vi "GO alertes Keller.vi"(5 "Numéro":u8) -> ()   [LabVIEW 2022 SP3]
uses:
  Enum/Enum s1.ctl
  Variables globales/Variable glob generale.vi
  Variables globales/Variable glob alertes Keller.vi
  Variables globales/Variable glob mails.vi
  Variables globales/Variable glob Keller.vi
panel:
  out "défaut max keller":bool
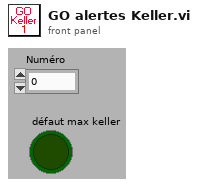
[diagram p1: front panel]
types:
  T1 = typedef "Enum s1.ctl" = enum16{"Alerte vide", "Alerte temperature min-max", "Alerte temperature ecart", "Alerte Keller", "Alerte compteur", "Alerte régulateurs"}
  T2 = cluster{"Alerte Keller":bool, "valeur alerte Keller":dbl, "Défaut Keller":bool, "Indices Keller à controler":i16[], "N°":u16}[]
  T3 = cluster{"Alerte Keller":bool, "valeur alerte Keller":dbl, "Défaut Keller":bool, "Indices Keller à controler":i16[], "N°":u16}
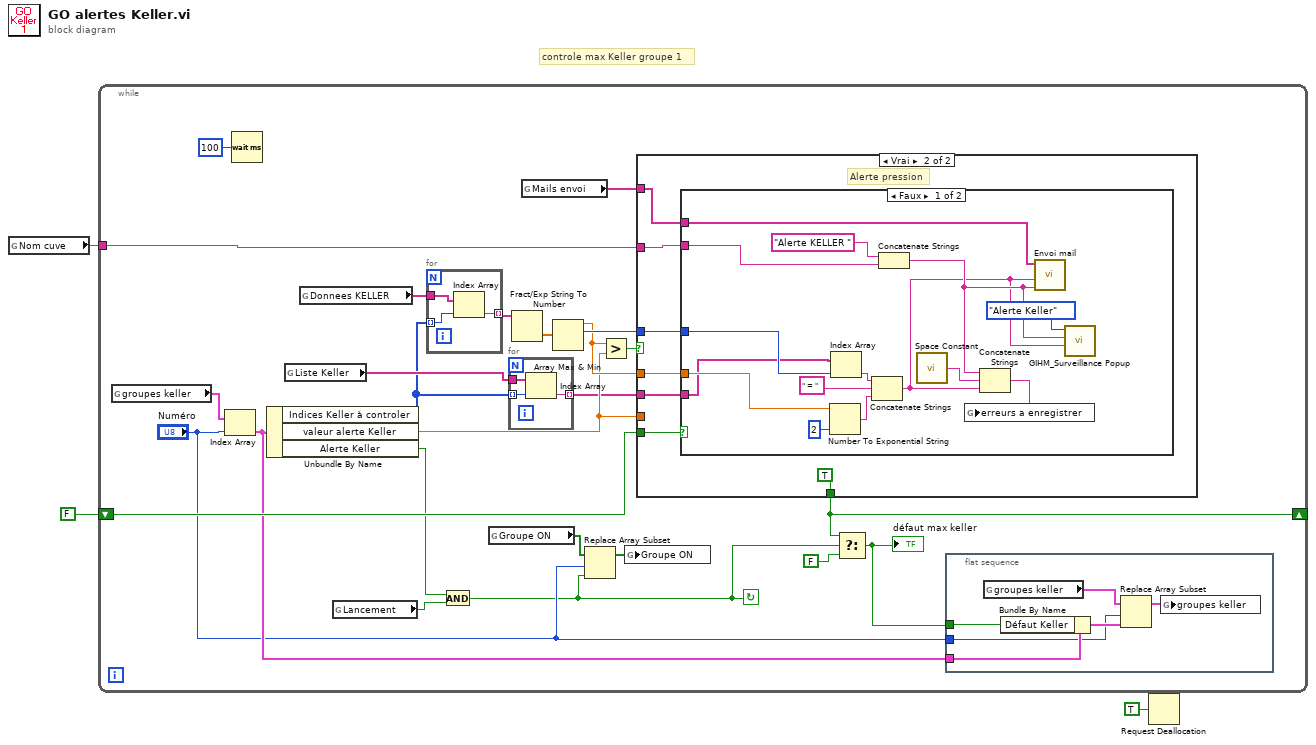
[diagram p0: block diagram]
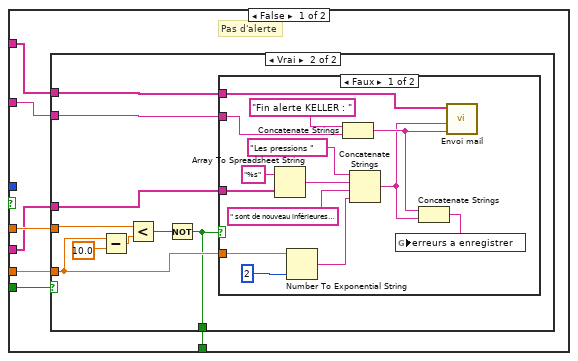
[diagram p2: hidden frame]
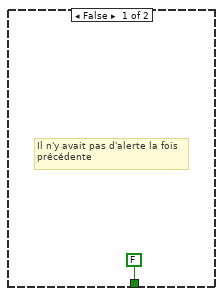
[diagram p3: hidden frame]
diagram:
  # "controle max Keller groupe 1"
  n1 = global read "Variable glob generale.vi" "Nom cuve"() -> (w2:string)
  n2 = while {
    tunnel: w2 -> [w26]
    shift-right: [w17] -> _
    shift-left: FALSE -> [w25]
    stop <- w5 continue-if-true
    n3 = global read "Variable glob alertes Keller.vi" "groupes keller"() -> (w14:T2)
    n4 = Index Array(array=w14, index="Numéro") -> (element=w15:T3)
    n5 = Wait (ms)(milliseconds to wait=u32 100 ("attente (ms)")) -> ()  [unwired: 1 out]
    n6 = Unbundle By Name(w15) -> ("Indices Keller à controler"=w11:i16[], "valeur alerte Keller"=w16:dbl, "Alerte Keller"=w9:bool)
    n7 = global read "Variable glob alertes Keller.vi" "Liste Keller"() -> (w12:string[])
    n8 = global read "Variable glob Keller.vi" "Donnees KELLER"() -> (w22:string[])
    n9 = global read "Variable glob generale.vi" "Lancement"() -> (w19:bool)
    n10 = for {
      tunnel: w22 -> [w92]
      tunnel: w11 -> [w93] mode=indexing
      tunnel: [w91] -> w28 mode=indexing
      n11 = Index Array(array=w92, index=w93) -> (element=w91:string)
    }
    n12 = And(x=w9, y=w19) -> (x .and. y?=w5:bool)
    n13 = global read "Variable glob alertes Keller.vi" "Groupe ON"() -> (w7:bool[])
    n14 = for {
      tunnel: w12 -> [w37]
      tunnel: w11 -> [w36] mode=indexing
      tunnel: [w35] -> w10 mode=indexing
      n15 = Index Array(array=w37, index=w36) -> (element=w35:string)
    }
    n16 = Fract/Exp String To Number(string=w28) -> (number=w20:dbl[])  [unwired: 3 in, 1 out]
    n17 = global read "Variable glob mails.vi" "Mails envoi"() -> (w8:string[])
    n18 = Array Max & Min(array=w20) -> (max value=w23:dbl, max index (indices)=w24:i32)  [unwired: 2 out]
    n19 = Replace Array Subset(array=w7, new element=w5, index="Numéro") -> (w4:bool[])
    n20 = Greater?(x=w23, y=w16) -> (0:w21:bool)
    n21 = global write "Variable glob alertes Keller.vi" "Groupe ON"(w4) -> ()
    n22 = case shown="Vrai" w21 {
      tunnel: w26 -> [w44 w75]
      tunnel: w25 -> [w42 w74]
      tunnel: w24 -> [_ w73]
      tunnel: w23 -> [w40 w72]
      tunnel: w16 -> [w43 _]
      tunnel: w8 -> [w41 w71]
      tunnel: [w39 TRUE] -> w17
      tunnel: w10 -> [w38 w69]
      frame False {
        # "Pas d'alerte"
        n23 = case shown="Vrai" w42 {
          tunnel: w43 -> [_ w48]
          tunnel: w44 -> [_ w53]
          tunnel: w41 -> [_ w54]
          tunnel: w40 -> [_ w52]
          tunnel: [FALSE w47] -> w39
          tunnel: w38 -> [_ w46]
          frame False {
            # "Il n'y avait pas d'alerte la fois\nprécédente"
          }
          frame True {
            n24 = Subtract(x=w48, y=10.0 ("x")) -> (x-y=w51:dbl)
            n25 = Less?(x=w52, y=w51) -> (x < y?=w50:bool)
            n26 = Not(x=w50) -> (.not. x?=w47:bool)
            n27 = case shown="Faux" w47 {
              tunnel: w48 -> [w68 _]
              tunnel: w54 -> [w65 _]
              tunnel: w53 -> [w64 _]
              tunnel: w46 -> [w61 _]
              frame False {
                n28 = Array To Spreadsheet String(array=w61, 3:"%s" ("chaîne de format")) -> (spreadsheet string=w58:string)  [unwired: 1 in]
                n29 = Number To Exponential String(number=w68, precision (6)=i16 2 ("précision (6)")) -> (E-format string=w55:string)  [unwired: 2 in]
                n30 = Concatenate Strings("Fin alerte KELLER : " ("subject ([No Subject])"), w64) -> (w62:string)
                n31 = Concatenate Strings("Les pressions ", w58, " sont de nouveau inférieures à ", w55) -> (w56:string)
                n32 = Concatenate Strings(w62, w56) -> (w63:string)
                n33 = global write "Variable glob generale.vi" "erreurs a enregistrer"(w63) -> ()
                n34 = call "Envoi mail.vi"("Objet"=w62, "Message"=w56, "Mail liste"=w65) -> ()  [unwired: 3 in]
              }
              frame True {
              }
            }
          }
        }
      }
      frame True {
        # "Alerte pression"
        n35 = case shown="Faux" w74 {
          tunnel: w75 -> [w82 _]
          tunnel: w73 -> [w87 _]
          tunnel: w72 -> [w86 _]
          tunnel: w71 -> [w83 _]
          tunnel: w69 -> [w81 _]
          frame False {
            n36 = Number To Exponential String(number=w86, precision (6)=i16 2 ("précision (6)")) -> (E-format string=w89:string)  [unwired: 2 in]
            n37 = Index Array(array=w81, index=w87) -> (element=w88:string)
            n38 = Concatenate Strings(w88, " = " ("chaîne"), w89) -> (w77:string)
            n39 = Concatenate Strings("Alerte KELLER " ("subject ([No Subject])"), w82) -> (w78:string)
            n40 = call <vilib>:"Space Constant.vi"() -> ("String"=w79:string)
            n41 = Concatenate Strings(w78, w79, w77) -> (w80:string)
            n42 = global write "Variable glob generale.vi" "erreurs a enregistrer"(w80) -> ()
            n43 = call "Envoi mail.vi"("Objet"=w78, "Message"=w77, "Mail liste"=w83) -> ()  [unwired: 3 in]
            n44 = call "GIHM_Surveillance Popup.vi"("Message"=w77, "Problème observé"=w78, "Type problème"=Enum_s1."Alerte Keller") -> ()  [unwired: 2 in, 1 out]
          }
          frame True {
            # "L'alerte était déjà présente"
          }
        }
      }
    }
    n45 = Select(t=w17, s=w5, f=FALSE ("cas faux")) -> (s? t:f=w13:bool)
    "défaut max keller" <- w13
    n46 = flat-sequence {
      tunnel: w15 -> [w34]
      tunnel: "Numéro" -> [w31]
      tunnel: w13 -> [w30]
      frame #0 {
        n47 = global read "Variable glob alertes Keller.vi" "groupes keller"() -> (w29:T2)
        n48 = Bundle By Name(cluster=w34, "Défaut Keller"=w30) -> (w33:T3)
        n49 = Replace Array Subset(array=w29, new element=w33, index=w31) -> (w32:T2)
        n50 = global write "Variable glob alertes Keller.vi" "groupes keller"(w32) -> ()
      }
    }
  }
  n51 = Request Deallocation(TRUE ("flag")) -> ()
